vi "Variant_ExtractClusterElements.vi"(11 "Cluster":variant) -> (1 "name":string, 2 "Elements":variant[](array[variant]), 3 "Cluster dup":variant)   [LabVIEW 2013, in "OpenVariant.lvlib"]
uses:
  OpenVariant.lvlib
  TypeDescriptor/TypeDescriptor_GetPString.vi
  TypeDescriptor/OpenDescriptor.lvlib
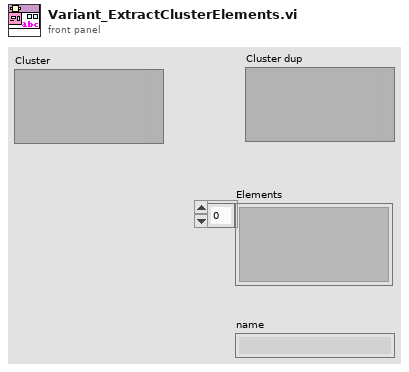
[diagram p1: front panel]
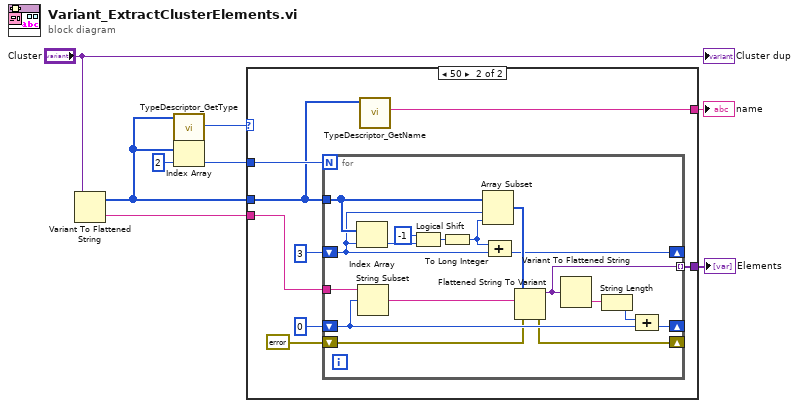
[diagram p0: block diagram]
diagram:
  n1 = Variant To Flattened String(Variant="Cluster") -> (data string=w8:string, 1:w2:i16[])
  n2 = call "TypeDescriptor_GetType.vi"("type descriptor"=w2) -> ("Type"=w1:u8)  [unwired: 9 in, 1 out]
  n3 = Index Array(array=w2, index=2) -> (element=w3:i16)
  n4 = case shown="50" w1 {
    tunnel: w8 -> [_ w16]
    tunnel: [_ w13] -> w7
    tunnel: [_ w12] -> w5
    tunnel: w3 -> [_ w10]
    tunnel: w2 -> [_ w9]
    frame Default {
      # "Not a cluster"
    }
    frame 80 {
      n5 = for {
        N: w10 -> [_]
        tunnel: w9 -> [w23]
        shift-right: [w28] -> _
        shift-left: 0 -> [w29]
        tunnel: w16 -> [w33]
        tunnel: [w27] -> w13 mode=indexing
        shift-right: [w25] -> _
        shift-left: errorcluster {"status"=FALSE, "code"=0, "source"=""} ("error out") -> [w26]
        shift-right: [w20] -> _
        shift-left: 3 -> [w19]
        n6 = Index Array(array=w23, index=w19) -> (element=w22:i16)
        n7 = String Subset(string=w33, offset (0)=w29) -> (substring=w32:string)  [unwired: 1 in]
        n8 = Logical Shift(y=i16 -1, x=w22) -> (x << y=w18:i16)
        n9 = To Long Integer(number=w18) -> (32bit integer=w17:i32)
        n10 = Array Subset(array=w23, index=w19, length=w17) -> (w24:i16[])
        n11 = Compound Arithmetic op=ADD(w17, w19) -> (w20:i32)
        n12 = Flattened String To Variant(4:w26, 6:w32, 7:w24) -> (0:w25:errorcluster, 3:w27:variant)
        n13 = Variant To Flattened String(Variant=w27) -> (data string=w31:string)  [unwired: 1 out]
        n14 = String Length(string=w31) -> (length=w30:i32)
        n15 = Compound Arithmetic op=ADD(w30, w29) -> (w28:i32)
      }
      n16 = call "TypeDescriptor_GetName.vi"("type descriptor"=w9) -> ("name"=w12:string)  [unwired: 8 in, 2 out]
    }
  }
  "Elements" <- w7
  "name" <- w5
  "Cluster dup" <- "Cluster"
